vi "Sim_Main.vi"(8 "error in (no error)":errorcluster={"status"=FALSE, "code"=0, "source"="\"\""}, 9 "current_ms":i64, 10 "pressure_target":dbl=150.0, 11 "time_advance_ms":i64=10) -> (0 "error out":errorcluster={"status"=FALSE, "code"=0, "source"="\"\""}, 1 "plant_power_kW":dbl, 2 "plant_pressure":dbl, 3 "sim_time_ms":i64)   [LabVIEW 2026]
doc: "INTENT: Top-level simulation executive coordinating simulated clock, VTU plant dynamics, and simulated I/O."
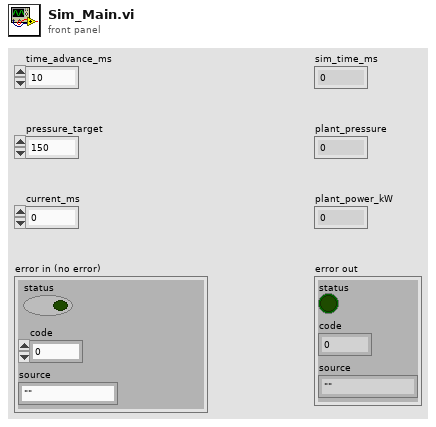
[diagram p1: front panel]
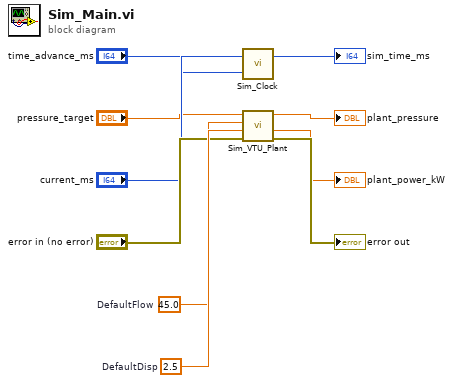
[diagram p0: block diagram]
diagram:
  w6 = 2.5  # DefaultDisp
  w5 = 45.0  # DefaultFlow
  n1 = call "Sim_Clock.vi"("advance_ms"="time_advance_ms", "current_ms"="current_ms") -> ("next_ms"=→"sim_time_ms":i64)  [unwired: 1 out]
  n2 = call "Sim_VTU_Plant.vi"("error in (no error)"="error in (no error)", "displacement_sp"=w6, "flow_sp"=w5, "pressure_sp"="pressure_target") -> ("error out"=→"error out":errorcluster, "act_power_kW"=→"plant_power_kW":dbl, "act_pressure"=→"plant_pressure":dbl)  [unwired: 4 in, 1 out]
